vi "Plugin_Cancel.vi"(8 "error in (no error)":errorcluster={"status"=FALSE, "code"=0, "source"="\"\""}, 10 "reason":string, 11 "Instance ID":string) -> (0 "error out":errorcluster={"status"=FALSE, "code"=0, "source"="\"\""}, 2 "status ok":bool, 3 "Cancel result":string)   [LabVIEW 2026]
doc: "INTENT: Request cooperative cancellation. LOGIC: Signal worker cancel, revoke hardware permissions immediately, mark incomplete on expiration."
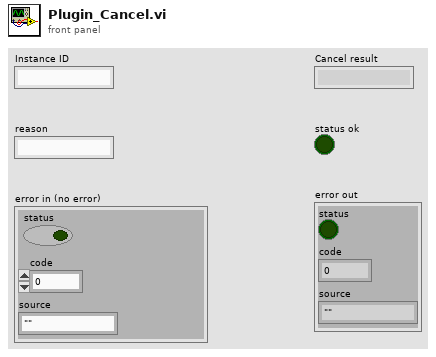
[diagram p1: front panel]
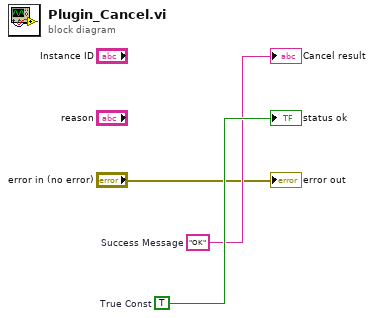
[diagram p0: block diagram]
diagram:
  w3 = TRUE  # True Const
  w2 = "OK"  # Success Message
  "Cancel result" <- w2
  "status ok" <- w3
  "error out" <- "error in (no error)"
